vi "Stop Core.vi"(10 "final error code":i32 caption="最终错误代码", 11 "Input Operator in":refnum<class "ControlPanel.lvclass"> caption="操作者输入") -> (3 "Input Operator out":refnum<class "ControlPanel.lvclass"> caption="操作者输出")   [LabVIEW 2014, in "ControlPanel.lvlib" / "ControlPanel.lvclass"]
doc: "(<B>文件名</B>：Actor Framework.lvlib:Actor.lvclass:Stop Core.vi)\n\n定义停止前操作者的动作。使用<B>最终错误代码</B>输入判断操作者是否在出错时关闭。\n\n默认情况下，该方法不执行任何动作。子孙类重写该方法，定义出错时的操作，例如，关闭操作者核心方法初始的进程。"
uses:
  ControlPanel.lvclass
  ControlPanel.lvclass/ControlPanel.ctl
  <vilib>/Utility/xml.llb/Write to XML File.vi
  Wrapper_lib/zsActor/ActorWrapper.lvclass
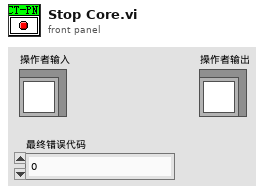
[diagram p1: front panel]
types:
  T1 = typedef "P3AT_Current.ctl" = cluster{"max_vel":dbl, "max_rot":dbl, "now_pose_X":dbl, "now_pose_Y":dbl, "now_pose_Rot_deg":dbl, "Control_Mode":enum32{"Joy", "Map", "Voice", "Input", "Undefined"}}
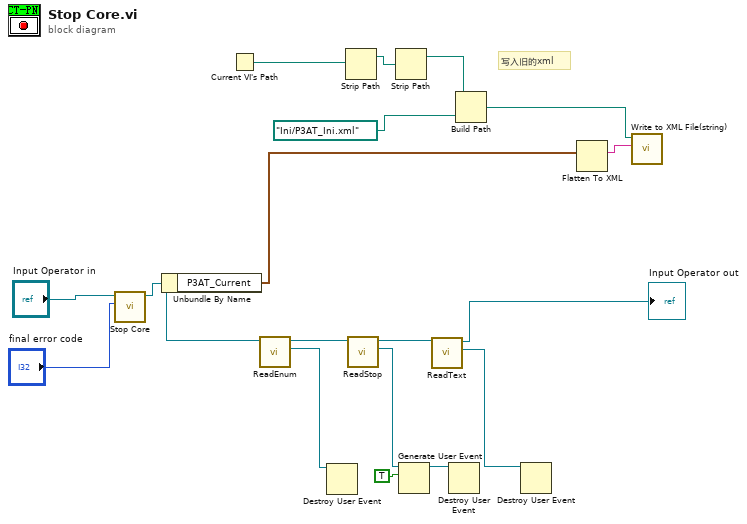
[diagram p0: block diagram]
diagram:
  # "写入旧的xml"
  n1 = call-parent "Stop Core.vi"("final error code"="final error code", "Actor in"="Input Operator in") -> ("Actor out"=w10:refnum<class "ControlPanel.lvclass">)  [unwired: 9 in]
  n2 = Unbundle By Name(w10) -> ("P3AT_Current"=w1:T1)
  n3 = Current VI's Path() -> (path=w11:path)
  n4 = call-dynamic "ReadEnum.vi"("zsActor输入"=w10) -> ("Enum"=w4:refnum<user-event>, "zsActor输出"=w9:refnum<class "ControlPanel.lvclass">)  [unwired: 8 in, 1 out]
  n5 = Destroy User Event(user event=w4) -> ()  [unwired: 1 in, 1 out]
  n6 = Strip Path(path=w11) -> (stripped path=w15:path)  [unwired: 1 out]
  n7 = call-dynamic "ReadStop.vi"("zsActor输入"=w9) -> ("Stop"=w3:refnum<user-event>, "zsActor输出"=w8:refnum<class "ControlPanel.lvclass">)  [unwired: 8 in, 1 out]
  n8 = Strip Path(path=w15) -> (stripped path=w14:path)  [unwired: 1 out]
  n9 = Generate User Event(user event=w3, event data cluster=TRUE ("event data")) -> (user event out=w5:refnum<user-event>)  [unwired: 2 in, 1 out]
  n10 = call-dynamic "ReadText.vi"("zsActor输入"=w8) -> ("Text"=w2:refnum<user-event>, "zsActor输出"=→"Input Operator out":refnum<class "ControlPanel.lvclass">)  [unwired: 8 in, 1 out]
  n11 = Destroy User Event(user event=w5) -> ()  [unwired: 1 in, 1 out]
  n12 = Build Path(base path=w14, name or relative path=path "Ini/P3AT_Ini.xml" ("拆分的路径")) -> (appended path=w12:path)
  n13 = Destroy User Event(user event=w2) -> ()  [unwired: 1 in, 1 out]
  n14 = Flatten To XML(anything=w1) -> (xml string=w16:string)
  n15 = call-poly <vilib>:"Write to XML File(string).vi"("XML Input"=w16, "XML File Path"=w12) -> ()  [unwired: 3 in, 7 out]
